vi "set Marker State.vi"(7 "Marker Mode":T1, 8 "error in (no error)":errorcluster, 9 "trace index":i32, 10 "Marker Index":i32, 11 "FSV-40N in":refnum<class "FSV-40N.lvclass">) -> (0 "error out":errorcluster, 3 "FSV-40N out":refnum<class "FSV-40N.lvclass">)   [LabVIEW 2023, in "Spectrum Analyzer.lvlib" / "FSV-40N.lvclass"]
uses:
  FSV-40N.lvclass
  FSV-40N.lvclass/FSV-40N.ctl
  TYPE DEFINITION/TYPE Marker Control Mode.ctl
  Spectrum Analyzer.lvlib
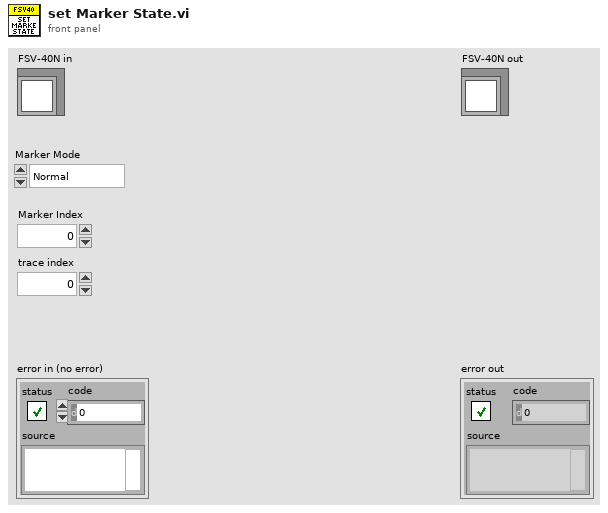
[diagram p1: front panel]
types:
  T1 = typedef "Spectrum Analyzer.lvlib/TYPE Marker Control Mode.ctl" = enum16{"Normal", "Delta", "Off"}
  T2 = typedef "Spectrum Analyzer.lvlib/TYPE Marker Type Map.ctl" = map{i32, T1}
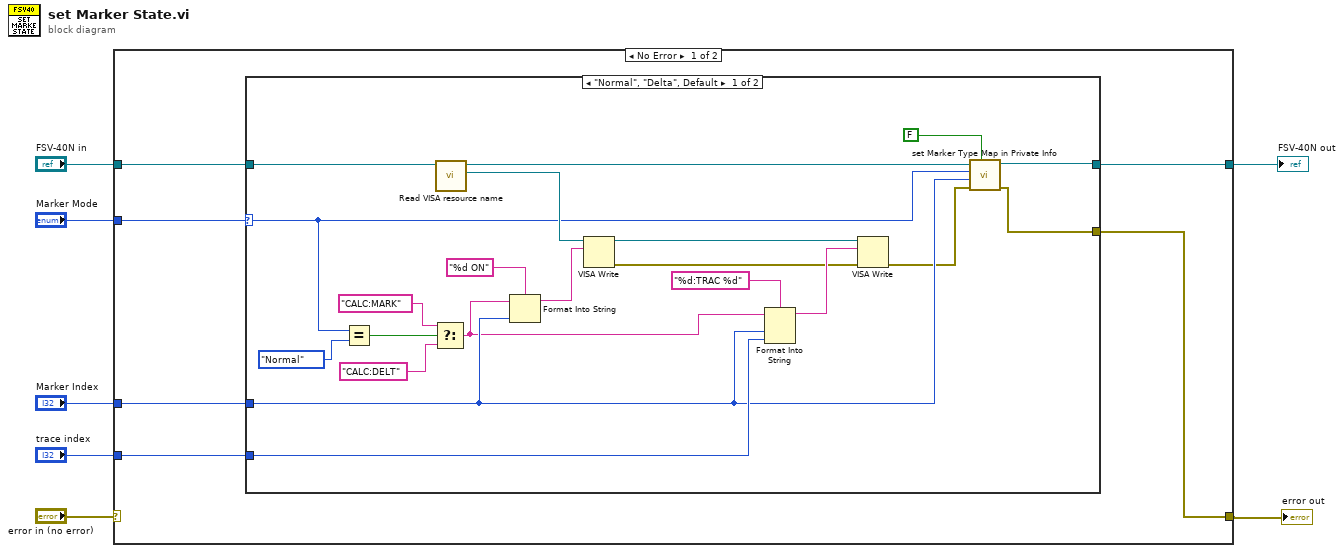
[diagram p0: block diagram]
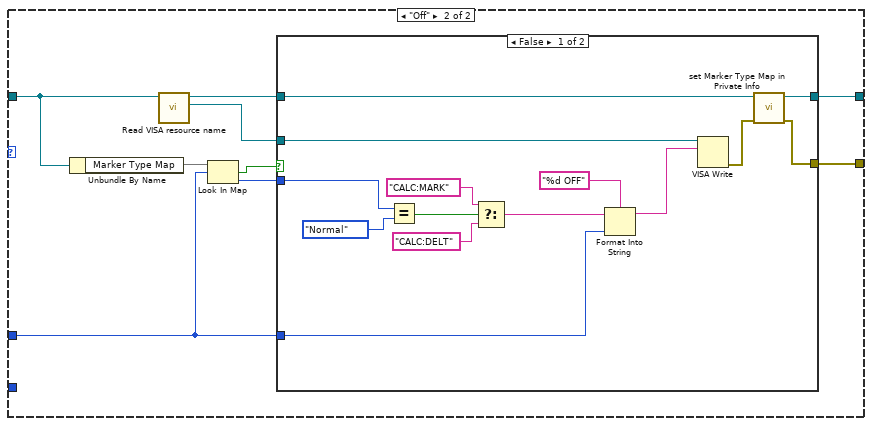
[diagram p2: hidden frame]
diagram:
  n1 = case shown="No Error" "error in (no error)" {
    selector: "error in (no error)" -> [_ w59]
    tunnel: "FSV-40N in" -> [w13 w60]
    tunnel: [w9 w60] -> w6
    tunnel: [w8 w59] -> w1
    tunnel: "Marker Mode" -> [w12 _]
    tunnel: "Marker Index" -> [w11 _]
    tunnel: "trace index" -> [w10 _]
    frame No Error {
      n2 = case shown="\"Normal\", \"Delta\", Default" w12 {
        selector: w12 -> [w14 _]
        tunnel: w13 -> [w22 w41]
        tunnel: w11 -> [w25 w39]
        tunnel: w10 -> [w26 _]
        tunnel: [w28 w43] -> w9
        tunnel: [w23 w36] -> w8
        frame "Normal", "Delta", Default {
          n3 = Equal?(x=w14, y=TYPE_Marker_Control_Mode."Normal") -> (x = y?=w18:bool)
          n4 = Select(t="CALC:MARK" ("initial string"), s=w18, f="CALC:DELT" ("initial string")) -> (s? t:f=w15:string)
          n5 = call "Read VISA resource name.vi"("FSV-40N in"=w22) -> ("VISA resource name"=w21:refnum<visa-resource-name>, "FSV-40N out"=w20:refnum<class "FSV-40N.lvclass">)  [unwired: 8 in, 1 out]
          n6 = Format Into String(format string="%d ON", initial string=w15, w25) -> (resulting string=w31:string)  [unwired: 1 in, 1 out]
          n7 = VISA Write(VISA resource name=w21, write buffer=w31) -> (VISA resource name out=w30:refnum<visa-resource-name>, error out=w29:errorcluster)  [unwired: 1 in, 1 out]
          n8 = Format Into String(format string="%d:TRAC %d", initial string=w15, w25, w26) -> (resulting string=w33:string)  [unwired: 1 in, 1 out]
          n9 = VISA Write(VISA resource name=w30, write buffer=w33, error in (no error)=w29) -> (error out=w24:errorcluster)  [unwired: 2 out]
          n10 = call "set Marker Type Map in Private Info.vi"("All Off?"=FALSE, "error in (no error)"=w24, "Marker Index"=w25, "Marker Mode"=w14, "FSV-40N in"=w20) -> ("error out"=w23:errorcluster, "FSV-40N out"=w28:refnum<class "FSV-40N.lvclass">)  [unwired: 5 in]
        }
        frame "Off" {
          n11 = Unbundle By Name(w41) -> ("Marker Type Map"=w40:T2)
          n12 = call "Read VISA resource name.vi"("FSV-40N in"=w41) -> ("VISA resource name"=w35:refnum<visa-resource-name>, "FSV-40N out"=w42:refnum<class "FSV-40N.lvclass">)  [unwired: 8 in, 1 out]
          n13 = Look In Map(map=w40, key=w39) -> (key not found?=w37:bool, value=w38:T1)  [unwired: 1 in]
          n14 = case shown="False" w37 {
            tunnel: [w55 w58] -> w43
            tunnel: w42 -> [w54 w58]
            tunnel: w39 -> [w53 _]
            tunnel: w38 -> [w52 _]
            tunnel: [w46 _] -> w36
            tunnel: w35 -> [w44 _]
            frame False {
              n15 = Equal?(x=w52, y=TYPE_Marker_Control_Mode."Normal") -> (x = y?=w50:bool)
              n16 = Select(t="CALC:MARK" ("initial string"), s=w50, f="CALC:DELT" ("initial string")) -> (s? t:f=w47:string)
              n17 = Format Into String(format string="%d OFF", initial string=w47, w53) -> (resulting string=w56:string)  [unwired: 1 in, 1 out]
              n18 = VISA Write(VISA resource name=w44, write buffer=w56) -> (error out=w45:errorcluster)  [unwired: 1 in, 2 out]
              n19 = call "set Marker Type Map in Private Info.vi"("error in (no error)"=w45, "FSV-40N in"=w54) -> ("error out"=w46:errorcluster, "FSV-40N out"=w55:refnum<class "FSV-40N.lvclass">)  [unwired: 8 in]
            }
            frame True {
            }
          }
        }
      }
    }
    frame Error {
    }
  }
  "error out" <- w1
  "FSV-40N out" <- w6
